vi "Interface.vi"() -> ()   [LabVIEW 2019, in "Operation Interface.lvclass"]
uses:
  Operation Interface.lvclass
  Robot/Universal Robot/Universal Robot.lvclass
  C:/_Code/Development/Sub-Zero Functional Test/standard hardware/Universal Robots/UR LabVIEW Interface/Classes/Application/Application Interfaces/Application Interface/Application Interface.lvclass
  Operation Interface.lvclass/Operation Interface.ctl
  Application Interface/FGVAction.ctl
  Application.lvclass
  Application Interface/Application Interface.lvclass
panel:
  out "Robot Mode":string
  out "robotModeColor":u32(colorbox)
  out "Operational Mode":string
  in  "powerOn":bool
  in  "brakeRelease":bool
  out "Safety Status":string
  out "safetyStatusColor":u32(colorbox)
  in  "restartSafety":bool
  in  "unlockProtectiveStop":bool
  in  "shutdownRobot":bool
  in  "sample rate (ms)":i32
  in  "interface":refnum<class "Operation Interface.lvclass">
  in  "robot":refnum<class "Universal Robot.lvclass">
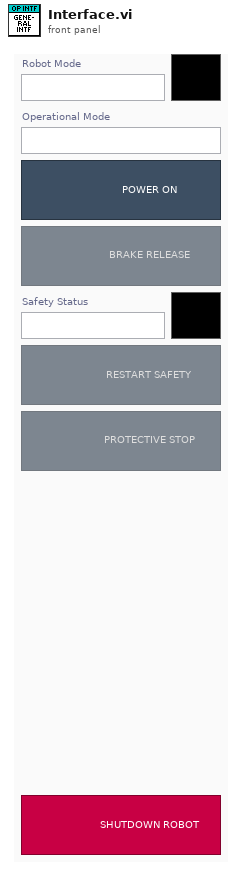
[diagram p1: front panel]
types:
  T1 = typedef "Universal Robot.lvclass/RobotStatus.ctl" = cluster{"Robot Mode":T2, "Operational Mode":T3, "Safety Status":T4, "Remote Control":bool}
  T2 = typedef "Universal Robot.lvclass/RobotMode.ctl" = enum16{"INVALID", "NO_CONTROLLER", "DISCONNECTED", "CONFIRM_SAFETY", "BOOTING", "POWER_OFF", "POWER_ON", "IDLE", "BACKDRIVE", "RUNNING"}
  T3 = typedef "Universal Robot.lvclass/OperationalMode.ctl" = enum16{"NONE", "MANUAL", "AUTOMATIC"}
  T4 = typedef "Universal Robot.lvclass/SafetyStatus.ctl" = enum16{"INVALID", "NORMAL", "REDUCED", "PROTECTIVE_STOP", "RECOVERY", "SAFEGUARD_STOP", "SYSTEM_EMERGENCY_STOP", "ROBOT_EMERGENCY_STOP", "VIOLATION", "FAULT", "AUTOMATIC_MODE_SAFEGAURD_STOP", "SYSTEM_THREE_POSITION_ENABLING_STOP"}
  T5 = typedef "Application Interface.lvclass/FGVAction.ctl" = enum16{"Initialize", "Get Last Status", "Update Status"}
  T6 = typedef "Application.lvclass/FrontPanelControls.ctl" = cluster{"Operation Interface":refnum<vi>, "Program Interface":refnum<vi>, "Command Interface":refnum<vi>, "Socket Interface":refnum<vi>, "Error Interface":refnum<vi>}
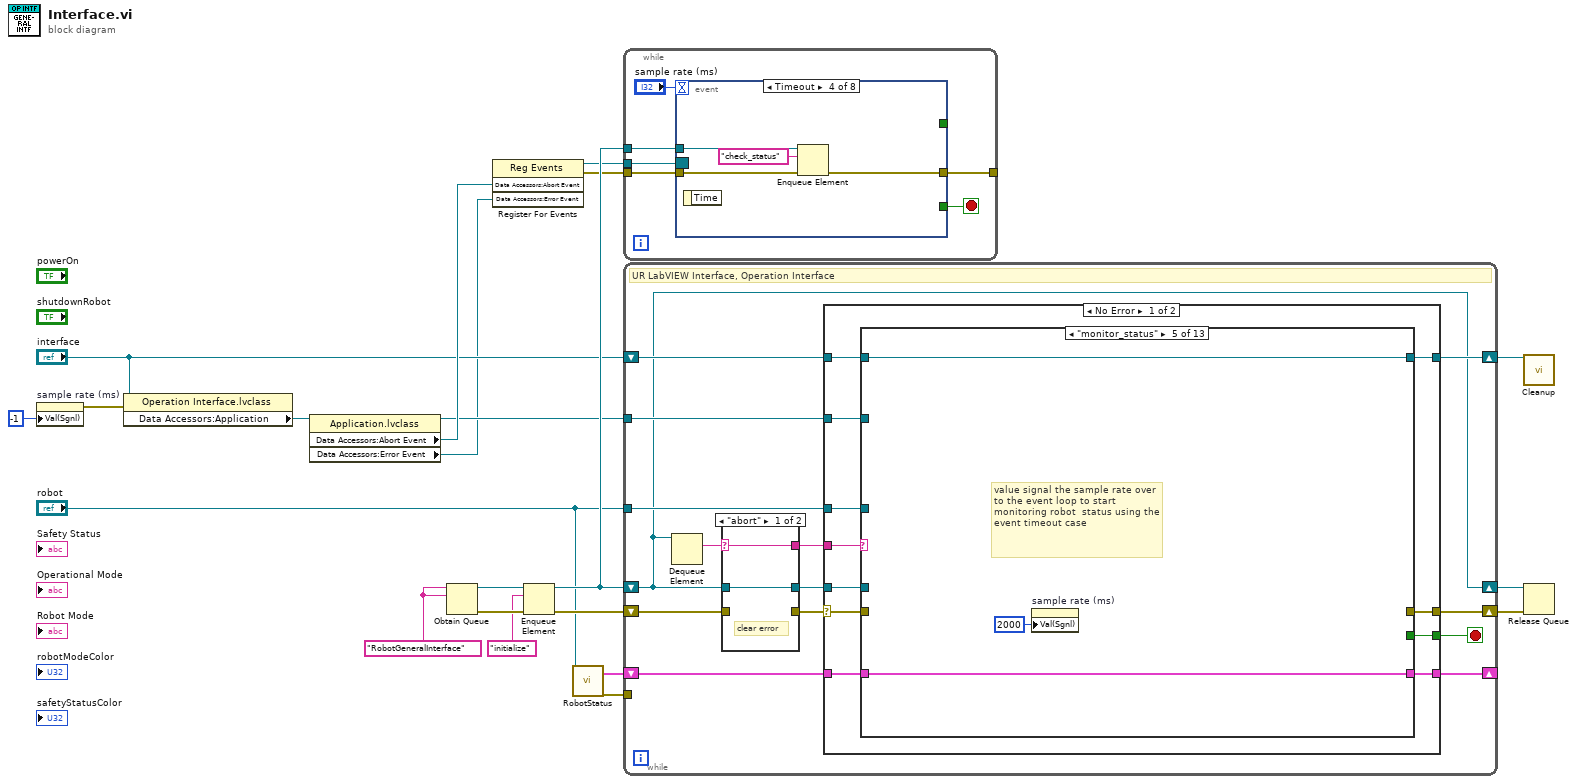
[diagram p0: block diagram]
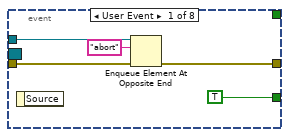
[diagram p2: hidden frame]
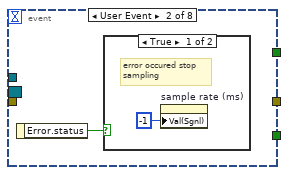
[diagram p3: hidden frame]
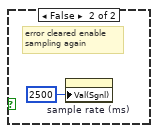
[diagram p4: hidden frame]
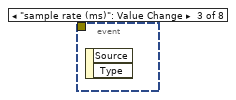
[diagram p5: hidden frame]
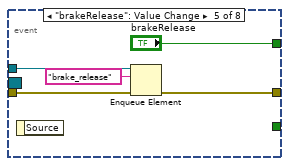
[diagram p6: hidden frame]
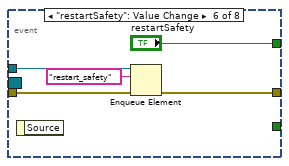
[diagram p7: hidden frame]
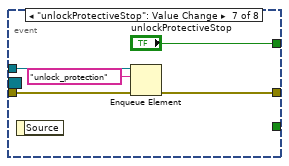
[diagram p8: hidden frame]
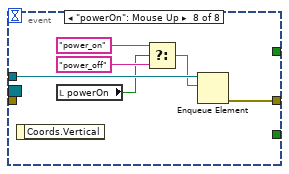
[diagram p9: hidden frame]
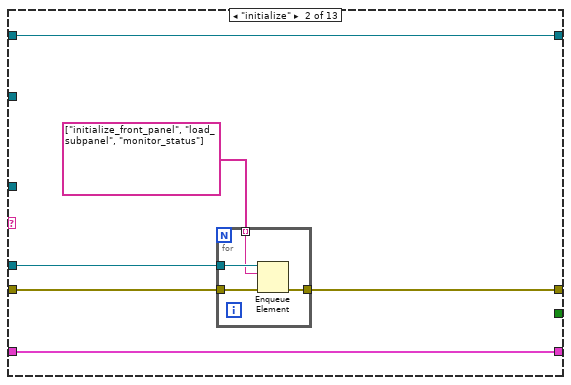
[diagram p12: hidden frame]
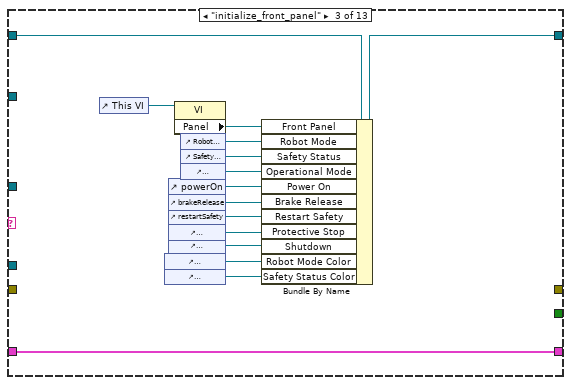
[diagram p13: hidden frame]
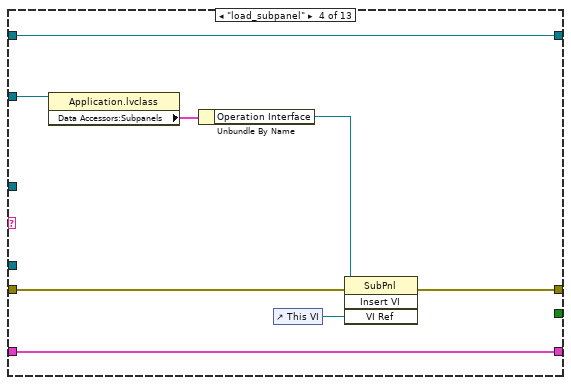
[diagram p14: hidden frame]
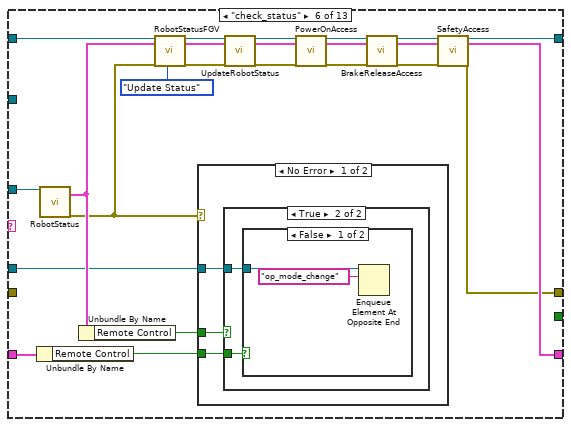
[diagram p15: hidden frame]
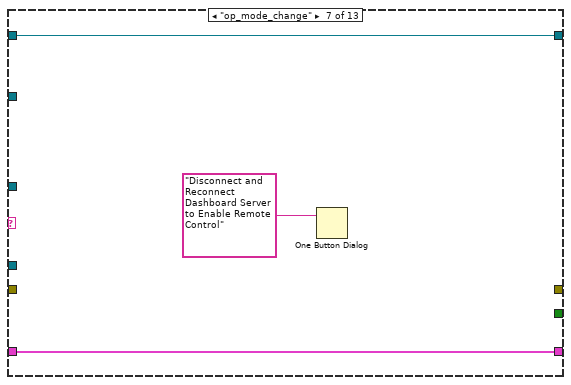
[diagram p19: hidden frame]
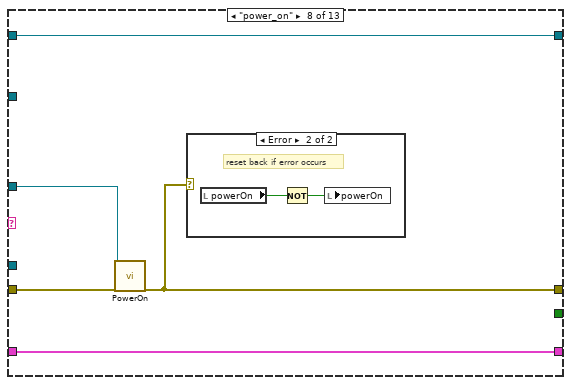
[diagram p20: hidden frame]
diagram:
  w16 = "RobotGeneralInterface" ("name (unnamed)")
  n1 = property on="sample rate (ms)" class="DigNum (strict)"("Val(Sgnl)"=-1 ("Value (Signaling)")) -> (error out=w4:errorcluster)  [unwired: 2 in, 1 out]
  n2 = property class="Operation Interface.lvclass"(reference="interface", error in=w4) -> ("Data Accessors:Application"=w11:refnum<class "Application.lvclass">)  [unwired: 2 out]
  n3 = property class="Application.lvclass"(reference=w11) -> (reference out=w9:refnum<class "Application.lvclass">, "Data Accessors:Abort Event"=w10:refnum<user-event>, "Data Accessors:Error Event"=w6:refnum<user-event>)  [unwired: 1 in, 1 out]
  n4 = Obtain Queue(name (unnamed)=w16, element data type=w16) -> (queue out=w20:refnum<queue>, error out=w21:errorcluster)  [unwired: 3 in, 1 out]
  n5 = register-events(w10, w6) -> (reference out=w12:refnum<event-registration>, error out=w13:errorcluster)  [unwired: 2 in]
  n6 = Enqueue Element(queue=w20, element="initialize", error in (no error)=w21) -> (queue out=w17:refnum<queue>, error out=w18:errorcluster)  [unwired: 1 in, 1 out]
  n7 = call-dynamic "RobotStatus.vi"("Universal Robot.lvclass in"="robot") -> ("Robot Status"=w2:T1, "error out"=w1:errorcluster)  [unwired: 16 in, 1 out]
  n8 = while {
    tunnel: w17 -> [w27]
    tunnel: w13 -> [w26]
    tunnel: w12 -> [w25]
    tunnel: [w24] -> _
    stop <- w23 stop-if-true
    n9 = event shown="[3] Timeout" {
      selector: w25 -> [_ _ _ _ _ _ _ _]
      dyn-events: _ -> [_ _ _ _ _ _ _ _]
      timeout: "sample rate (ms)" -> [_ _ _ _ _ _ _ _]
      tunnel: w27 -> [w32 _ _ w39 w44 w49 w54 w60]
      tunnel: w26 -> [w31 _ _ w38 w43 w48 w53 _]
      tunnel: [w30 _ _ w37 w42 w47 w52 w59] -> w24
      tunnel: [TRUE _ _ _ _ _ _ _] -> w23
      tunnel: [_ _ _ _ "brakeRelease" "restartSafety" "unlockProtectiveStop" _] -> _
      event User Event {
        n10 = event-data() -> ()  [unwired: 1 in, 1 out]
        n11 = Enqueue Element At Opposite End(queue=w32, element="abort", error in (no error)=w31) -> (error out=w30:errorcluster)  [unwired: 1 in, 2 out]
      }
      event User Event {
        n12 = event-data() -> ("Error.status"=w33:bool)  [unwired: 1 in]
        n13 = case shown="True" w33 {
          frame True {
            # "error occured stop\nsampling"
            n14 = property on="sample rate (ms)" class="DigNum (strict)"("Val(Sgnl)"=-1 ("Value (Signaling)")) -> ()  [unwired: 2 in, 2 out]
          }
          frame False {
            # "error cleared enable\nsampling again"
            n15 = property on="sample rate (ms)" class="DigNum (strict)"("Val(Sgnl)"=2500 ("Value (Signaling)")) -> ()  [unwired: 2 in, 2 out]
          }
        }
      }
      event "sample rate (ms)": Value Change {
        n16 = event-data() -> ()  [unwired: 1 in, 2 out]
      }
      event Timeout {
        n17 = event-data() -> ()  [unwired: 1 in, 1 out]
        n18 = Enqueue Element(queue=w39, element="check_status", error in (no error)=w38) -> (error out=w37:errorcluster)  [unwired: 1 in, 2 out]
      }
      event "brakeRelease": Value Change {
        n19 = event-data() -> ()  [unwired: 1 in, 1 out]
        n20 = Enqueue Element(queue=w44, element="brake_release", error in (no error)=w43) -> (error out=w42:errorcluster)  [unwired: 1 in, 2 out]
      }
      event "restartSafety": Value Change {
        n21 = event-data() -> ()  [unwired: 1 in, 1 out]
        n22 = Enqueue Element(queue=w49, element="restart_safety", error in (no error)=w48) -> (error out=w47:errorcluster)  [unwired: 1 in, 2 out]
      }
      event "unlockProtectiveStop": Value Change {
        n23 = event-data() -> ()  [unwired: 1 in, 1 out]
        n24 = Enqueue Element(queue=w54, element="unlock_protection", error in (no error)=w53) -> (error out=w52:errorcluster)  [unwired: 1 in, 2 out]
      }
      event "powerOn": Mouse Up {
        n25 = event-data() -> ()  [unwired: 1 in, 1 out]
        n26 = local read "powerOn"() -> (w55:bool)
        n27 = Select(t="power_on", s=w55, f="power_off") -> (s? t:f=w57:string)
        n28 = Enqueue Element(queue=w60, element=w57) -> (error out=w59:errorcluster)  [unwired: 2 in, 2 out]
      }
    }
  }
  n29 = while {
    shift-right: [w74] -> w14
    shift-left: w18 -> [w64]
    shift-right: [w62] -> w15
    shift-left: w17 -> [w62]
    tunnel: "robot" -> [w71]
    tunnel: w9 -> [w70]
    shift-right: [w69] -> w7
    shift-left: "interface" -> [w72]
    shift-right: [w68] -> _
    shift-left: w2 -> [w67]
    tunnel: w1 -> [_]
    stop <- w73 stop-if-true
    # "UR LabVIEW Interface, Operation Interface"
    n30 = Dequeue Element(queue=w62) -> (element=w66:string)  [unwired: 2 in, 3 out]
    n31 = case shown="\"abort\"" w66 {
      selector: w66 -> [w76 w79]
      tunnel: [w76 w79] -> w65
      tunnel: w64 -> [_ w78]
      tunnel: [_ w78] -> w63
      tunnel: w62 -> [w75 w77]
      tunnel: [w75 w77] -> w61
      frame "abort" {
        # "clear error"
      }
      frame Default {
      }
    }
    n32 = case shown="No Error" w63 {
      selector: w63 -> [w80 w202]
      tunnel: [w90 _] -> w74
      tunnel: [w89 _] -> w73
      tunnel: w72 -> [w88 w203]
      tunnel: w71 -> [w87 _]
      tunnel: w70 -> [w86 w201]
      tunnel: [w85 w203] -> w69
      tunnel: [w84 w204] -> w68
      tunnel: w67 -> [w83 w204]
      tunnel: w65 -> [w82 _]
      tunnel: w61 -> [w81 _]
      frame No Error {
        n33 = case shown="\"monitor_status\"" w82 {
          tunnel: w80 -> [w93 w97 _ w122 _ _ _ w167 w174 w181 w186 w191 w198]
          tunnel: w81 -> [_ w98 _ _ _ w130 _ _ _ _ _ _ _]
          tunnel: [w93 w96 _ w126 _ w131 _ w165 w172 w179 w184 w189 w197] -> w90
          tunnel: [_ _ _ _ _ _ _ _ _ _ _ _ TRUE] -> w89
          tunnel: w88 -> [w92 w99 w118 w124 w129 w146 w163 w166 w175 w182 w187 w192 w199]
          tunnel: w87 -> [_ _ _ _ _ w153 _ w168 w173 w180 w185 w190 _]
          tunnel: w86 -> [_ _ _ w123 _ _ _ _ _ _ _ _ w196]
          tunnel: [w92 w99 w117 w124 w129 w140 w163 w166 w175 w182 w187 w192 w199] -> w85
          tunnel: [w91 w94 w104 w119 w128 w136 w162 w164 w171 w178 w183 w188 w193] -> w84
          tunnel: w83 -> [w91 w94 w104 w119 w128 w139 w162 w164 w171 w178 w183 w188 w193]
          frame Default {
          }
          frame "initialize" {
            n34 = for {
              tunnel: w98 -> [w103]
              tunnel: w97 -> [w102]
              tunnel: [w101] -> w96
              tunnel: string[] ["initialize_front_panel", "load_subpanel", "monitor_status"] -> [w100] mode=indexing
              n35 = Enqueue Element(queue=w103, element=w100, error in (no error)=w102) -> (error out=w101:errorcluster)  [unwired: 1 in, 2 out]
            }
          }
          frame "initialize_front_panel" {
            n36 = control-ref of="This VI"() -> (w107:refnum<vi>)
            n37 = control-ref of="robotModeColor"() -> (w115:refnum<vi>)
            n38 = control-ref of="safetyStatusColor"() -> (w108:refnum<vi>)
            n39 = control-ref of="powerOn"() -> (w113:refnum<vi>)
            n40 = control-ref of="brakeRelease"() -> (w112:refnum<vi>)
            n41 = control-ref of="restartSafety"() -> (w111:refnum<vi>)
            n42 = control-ref of="unlockProtectiveStop"() -> (w110:refnum<vi>)
            n43 = control-ref of="shutdownRobot"() -> (w109:refnum<vi>)
            n44 = property class="VI"(reference=w107) -> ("Panel"=w106:refnum<vi>)  [unwired: 1 in, 2 out]
            n45 = control-ref of="Robot Mode"() -> (w116:refnum<vi>)
            n46 = control-ref of="Safety Status"() -> (w105:refnum<vi>)
            n47 = control-ref of="Operational Mode"() -> (w114:refnum<vi>)
            n48 = Bundle By Name(cluster=w118, "Front Panel"=w106, "Robot Mode"=w116, "Safety Status"=w105, "Operational Mode"=w114, "Power On"=w113, "Brake Release"=w112, "Restart Safety"=w111, "Protective Stop"=w110, "Shutdown"=w109, "Robot Mode Color"=w115, "Safety Status Color"=w108) -> (w117:refnum<class "Operation Interface.lvclass">)
          }
          frame "load_subpanel" {
            n49 = property class="Application.lvclass"(reference=w123) -> ("Data Accessors:Subpanels"=w121:T6)  [unwired: 1 in, 2 out]
            n50 = Unbundle By Name(w121) -> ("Operation Interface"=w120:refnum<vi>)
            n51 = control-ref of="This VI"() -> (w125:refnum<vi>)
            n52 = invoke class="SubPnl" method="Insert VI"(reference=w120, error in=w122, "VI Ref"=w125) -> (error out=w126:errorcluster)  [unwired: 1 in, 3 out]
          }
          frame "monitor_status" {
            # "value signal the sample rate over to the event loop to start monitoring robot  status using the event timeout case"
            n53 = property on="sample rate (ms)" class="DigNum (strict)"("Val(Sgnl)"=2000 ("Value (Signaling)")) -> ()  [unwired: 2 in, 2 out]
          }
          frame "check_status" {
            n54 = Unbundle By Name(w139) -> ("Remote Control"=w134:bool)
            n55 = call-dynamic "RobotStatus.vi"("Universal Robot.lvclass in"=w153) -> ("Robot Status"=w138:T1, "error out"=w132:errorcluster)  [unwired: 16 in, 1 out]
            n56 = Unbundle By Name(w138) -> ("Remote Control"=w135:bool)
            n57 = call "RobotStatusFGV.vi"("Application Interface in"=w146, "Robot Status in"=w138, "error in (no error)"=w132, "Action (Read)"=FGVAction."Update Status") -> ("Application Interface out"=w145:refnum<class "Operation Interface.lvclass">, "Robot Status out"=w137:T1, "error out"=w133:errorcluster)  [unwired: 13 in]
            n58 = case shown="No Error" w132 {
              tunnel: w135 -> [w156 _]
              tunnel: w134 -> [w155 _]
              tunnel: w130 -> [w154 _]
              frame No Error {
                n59 = case shown="True" w156 {
                  tunnel: w155 -> [_ w158]
                  tunnel: w154 -> [_ w157]
                  frame False {
                  }
                  frame True {
                    n60 = case shown="False" w158 {
                      tunnel: w157 -> [w160 _]
                      frame False {
                        n61 = Enqueue Element At Opposite End(queue=w160, element="op_mode_change") -> ()  [unwired: 2 in, 3 out]
                      }
                      frame True {
                      }
                    }
                  }
                }
              }
              frame Error {
              }
            }
            n62 = call "UpdateRobotStatus.vi"("Operation Interface in"=w145, "Robot Status"=w137, "error in (no error)"=w133) -> ("Operation Interface out"=w152:refnum<class "Operation Interface.lvclass">, "Robot Status Out"=w151:T1, "error out"=w150:errorcluster)  [unwired: 14 in]
            n63 = call "PowerOnAccess.vi"("Operation Interface in"=w152, "Robot Status"=w151, "error in (no error)"=w150) -> ("Operation Interface out"=w149:refnum<class "Operation Interface.lvclass">, "Robot Status Out"=w147:T1, "error out"=w148:errorcluster)  [unwired: 14 in]
            n64 = call "BrakeReleaseAccess.vi"("Operation Interface in"=w149, "Robot Status in"=w147, "error in (no error)"=w148) -> ("Operation Interface out"=w143:refnum<class "Operation Interface.lvclass">, "Robot Status out"=w141:T1, "error out"=w142:errorcluster)  [unwired: 14 in]
            n65 = call "SafetyAccess.vi"("Operation Interface in"=w143, "Robot Status In"=w141, "error in (no error)"=w142) -> ("Operation Interface out"=w140:refnum<class "Operation Interface.lvclass">, "Robot Status Out"=w136:T1, "error out"=w131:errorcluster)  [unwired: 14 in]
          }
          frame "op_mode_change" {
            n66 = One Button Dialog(message="Disconnect and Reconnect Dashboard Server to Enable Remote Control") -> ()  [unwired: 1 in, 1 out]
          }
          frame "power_on" {
            n67 = call-dynamic "PowerOn.vi"("Universal Robot.lvclass in"=w168, "error in (no error)"=w167) -> ("error out"=w165:errorcluster)  [unwired: 16 in, 1 out]
            n68 = case shown="Error" w165 {
              frame No Error {
              }
              frame Error {
                # "reset back if error occurs"
                n69 = local read "powerOn"() -> (w170:bool)
                n70 = Not(x=w170) -> (.not. x?=w169:bool)
                n71 = local write "powerOn"(w169) -> ()
              }
            }
          }
          frame "power_off" {
            n72 = call-dynamic "PowerOff.vi"("Universal Robot.lvclass in"=w173, "error in (no error)"=w174) -> ("error out"=w172:errorcluster)  [unwired: 16 in, 1 out]
            n73 = case shown="Error" w172 {
              frame No Error {
              }
              frame Error {
                # "reset back if error occurs"
                n74 = local read "powerOn"() -> (w177:bool)
                n75 = Not(x=w177) -> (.not. x?=w176:bool)
                n76 = local write "powerOn"(w176) -> ()
              }
            }
          }
          frame "brake_release" {
            n77 = call-dynamic "BrakeRelease.vi"("Universal Robot.lvclass in"=w180, "error in (no error)"=w181) -> ("error out"=w179:errorcluster)  [unwired: 16 in, 1 out]
          }
          frame "restart_safety" {
            n78 = call-dynamic "RestartSafety.vi"("Universal Robot.lvclass in"=w185, "error in (no error)"=w186) -> ("error out"=w184:errorcluster)  [unwired: 16 in, 1 out]
          }
          frame "unlock_protection" {
            n79 = call-dynamic "UnlockProtectiveStop.vi"("Universal Robot.lvclass in"=w190, "error in (no error)"=w191) -> ("error out"=w189:errorcluster)  [unwired: 16 in, 1 out]
          }
          frame "abort" {
            n80 = property class="Application.lvclass"(reference=w196) -> ("Data Accessors:Subpanels"=w195:T6)  [unwired: 1 in, 2 out]
            n81 = Unbundle By Name(w195) -> ("Operation Interface"=w194:refnum<vi>)
            n82 = invoke class="SubPnl" method="Remove VI"(reference=w194, error in=w198) -> (error out=w197:errorcluster)  [unwired: 1 in, 2 out]
          }
        }
      }
      frame Error {
        n83 = call "Generate Error.vi"("Application in"=w201, "error in (no error)"=w202) -> ()  [unwired: 17 in, 1 out]
      }
    }
  }
  n84 = call "Cleanup.vi"("Operation Interface in"=w7) -> ()  [unwired: 19 in]
  n85 = Release Queue(queue=w15, error in (no error)=w14) -> ()  [unwired: 1 in, 3 out]
